vi "Main Editor UI.vi"() -> ()   [LabVIEW 2015, in "SystemLink editor node.lvclass"]
doc: "This is the main view for configuration the behavior of a module in the DCAF standard editor."
uses:
  SystemLink editor node.lvclass
  <vilib>/NI/Configuration Framework/Node/NodeRef.ctl
  <vilib>/NI/Configuration Framework/Node/NISE_CEF_Node.lvclass
  <vilib>/NI/AMC/Message Queue.ctl
  <vilib>/NI/AMC/Message.ctl
  <vilib>/NI/Tools/Keyed Array/KeyedArray.ctl
  <vilib>/NI/Configuration Framework/Node/UserEventRef.ctl
  <vilib>/NI/Configuration Framework/Controls/EventCluster.ctl
  <vilib>/NI/DCAF UI Toolkit/Controls/Configure.ctl
  <vilib>/NI/DCAF UI Toolkit/Controls/Add.ctl
  <vilib>/NI/DCAF UI Toolkit/Controls/Remove.ctl
  <vilib>/NI/Configuration Framework/Node/StopEvent.ctl
  <vilib>/NI/Configuration Framework/Node/RefreshUIEvent.ctl
  <vilib>/NI/Configuration Framework/Node/CacheState.ctl
  <vilib>/NI/Configuration Framework/Node/NodeChangeEvent.ctl
  module/configuration/Permissions Enum.ctl
  <vilib>/NI/DCAF/Tag Editor Core/Table API/Available Tag Menu/channel action event.ctl
  <vilib>/NI/DCAF/Tag Editor Core/Table API/Available Tag Menu/dialog output action.ctl
  <vilib>/NI/Tag Bus Module Framework/channel/TBM channel.lvclass
  <vilib>/NI/Tag Bus/tag/tag descriptor.lvclass
  <vilib>/NI/DCAF/Tag Editor Core/Table API/Table Manager/Call Back Ref Type Def.ctl
  <vilib>/NI/DCAF/Tag Editor Core/Configuration Editor/Classes/Engine Parent/Engine Parent Editor Node.lvclass
  <vilib>/NI/DCAF/Tag Editor Core/Configuration Editor/Classes/Module editor node/module editor node.lvclass
  <vilib>/NI/DCAF UI Toolkit/Controls/Import.ctl
  <vilib>/NI/DCAF UI Toolkit/Controls/Export.ctl
  module/configuration/Data Tag Type.ctl
  <vilib>/NI/DCAF/Tag Editor Core/Table API/Table Manager/references.ctl
  module/configuration/SystemLink configuration.lvclass
  module/configuration/SystemLink configuration.lvclass/SystemLink configuration.ctl
  <vilib>/Utility/miscctls.llb/LVPositionTypeDef.ctl
  module/configuration/Read Connection Configuration.vi
  module/configuration/Read Prepend Minion ID.vi
  <vilib>/NI/Configuration Framework/serializable configuration/NISE_CEF_serializable configuration.lvclass
  <vilib>/NI/DCAF/Tag Editor Core/Table API/Listbox/Multi Column Listbox.lvclass
  <vilib>/NI/Configuration Framework/NISE_CEF_TreeControl.lvlib
  <vilib>/NI/Tools/Keyed Array/Tools_KeyedArray.lvlib
  <vilib>/NI/AMC/AMC.lvlib
  <vilib>/NI/DCAF/Tag Editor Core/Table API/Table Manager.lvlib
  <vilib>/NI/DCAF/Tag Editor Core/Table API/Table Manager/Table Manager.lvclass
  <vilib>/NI/DCAF UI Toolkit/Controls/DCAF UI Elements.lvlib
panel:
  in  "Data Type":T1
  in  "user event out":refnum<user-event>
  in  "Permissions":T2
  in  "node change":T3
  in  "cache state":T4
  in  "refresh UI":T5
  in  "stop event":T6
  in  "Tab Control":T7(tab)
  in  "PrependMinionID":bool=TRUE caption="Prepend Tags With Minion ID?"
  in  "Remove Button":T8
  in  "Add Button":T9
  in  "Table":i32(listbox)
  in  "settings":T10
  in  "Configuration":T11={"Configuration ID"="", "HTTP"={"Verify Server?"=TRUE, "Server URL"="", "CA Certificate File"="", "User Info"={"Username"="", "Password"=""}, "API Key"=""}}
  in  "Connection Type":T12(ring)
  in  "Export":T13
  in  "Import":T14
  in  "user event":T15
  in  "main queue":T16
  in  "node ref":T17
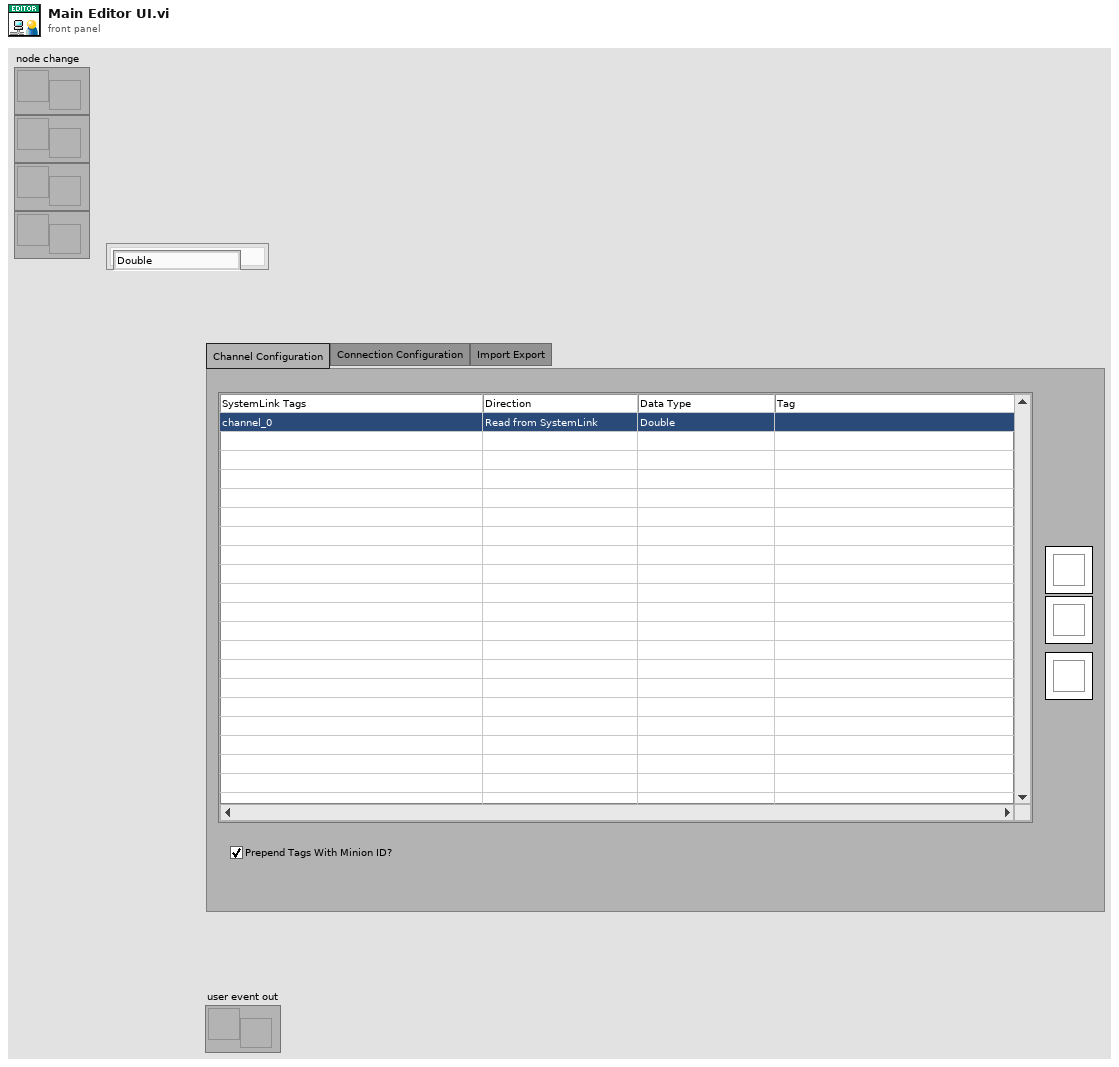
[diagram p1: front panel]
types:
  T1 = typedef "SystemLink configuration.lvclass/Data Tag Type.ctl" = enum16{"Double", "Single", "I32", "I16", "I8", "U64", "U32", "U16", "U8", "Boolean", "String", "Timestamp"}
  T2 = typedef "SystemLink configuration.lvclass/Permissions Enum.ctl" = enum16{"Read from SystemLink", "Write to SystemLink"}
  T3 = typedef "NISE_CEF_Node.lvclass/NodeChangeEvent.ctl" = refnum<user-event>
  T4 = typedef "NISE_CEF_Node.lvclass/CacheState.ctl" = refnum<user-event>
  T5 = typedef "NISE_CEF_Node.lvclass/RefreshUIEvent.ctl" = refnum<user-event>
  T6 = typedef "NISE_CEF_Node.lvclass/StopEvent.ctl" = refnum<user-event>
  T7 = enum32{"Channel Configuration", "Connection Configuration", "Import Export"}
  T8 = typedef "DCAF UI Elements.lvlib/Remove.ctl" = bool
  T9 = typedef "DCAF UI Elements.lvlib/Add.ctl" = bool
  T10 = typedef "DCAF UI Elements.lvlib/Configure.ctl" = bool
  T11 = cluster{"Configuration ID":string, "HTTP":cluster{"Verify Server?":bool, "Server URL":string, "CA Certificate File":string, "User Info":cluster{"Username":string, "Password":string}, "API Key":string}}
  T12 = enum16{"AMQP", "HTTP", "API Key (SystemLink Cloud)"}
  T13 = typedef "DCAF UI Elements.lvlib/Export.ctl" = bool
  T14 = typedef "DCAF UI Elements.lvlib/Import.ctl" = bool
  T15 = typedef "NISE_CEF_Node.lvclass/UserEventRef.ctl" = refnum<user-event>
  T16 = typedef "AMC.lvlib/Message Queue.ctl" = refnum<queue>
  T17 = typedef "NISE_CEF_Node.lvclass/NodeRef.ctl" = refnum<data-value>
  T18 = typedef "Table Manager.lvlib/Table Manager.lvclass/references.ctl" = cluster{"stop event":T6, "refresh UI":T5, "cache state":T4, "node change":T3, "user event out":refnum<user-event>, "main queue":T16, "user event":T15}
  T19 = typedef "LVPositionTypeDef.ctl" = cluster{"Left":i32, "Top":i32}
  T20 = typedef "Table Manager.lvlib/Table Manager.lvclass/object ref.ctl" = cluster{"engine":refnum<data-value>, "Node Ref":refnum<data-value>}
  T21 = typedef "Table Manager.lvlib/Column.lvclass/Column Descriptor.ctl" = cluster{"name":string, "caption":string, "Column Type":T22, "Params":string, "AutoSizeMode":i32, "FillWeight":sgl, "MinWidth":u32, "tooltip":string, "Enum Reference":refnum<vi>, "Channel suffix":string, "Read Only":bool, "Call Back VI":T23, "DT Dependency":i32, "name dependency":i32, "data type":T24, "Custom Column":refnum<class "Column.lvclass">}
  T22 = typedef "Table Manager.lvlib/Column.lvclass/Column Type.ctl" = enum16{"String", "Mapping", "Enum", "Custom"}
  T23 = typedef "Table Manager.lvlib/Table Manager.lvclass/Call Back Ref Type Def.ctl" = refnum<vi>
  T24 = typedef "tag bus.lvlib/tag descriptor.lvclass/Data Type.ctl" = enum16{"Double", "Single", "I64", "I32", "I16", "I8", "U64", "U32", "U16", "U8", "Boolean", "String", "Array of Double", "Array of Single", "Array of I64", "Array of I32", "Array of I16", "Array of I8", "Array of U64", "Array of U32", "Array of U16", "Array of U8", "Array of Boolean", "Array of String"}
  T25 = typedef "SystemLink configuration.lvclass/Connection Configuration.ctl" = cluster{"Connection Type":T26, "AMQP":cluster{"Configuration ID":string}, "HTTP":cluster{"Verify Server?":bool, "Server URL":string, "CA Certificate File":string, "User Info":cluster{"Username":string, "Password":string}, "API Key":string}}
  T26 = typedef "SystemLink configuration.lvclass/Connection Type.ctl" = enum16{"AMQP", "HTTP", "API Key (SystemLink Cloud)"}
  T27 = cluster{"Verify Server?":bool, "Server URL":string, "CA Certificate File":string, "User Info":cluster{"Username":string, "Password":string}, "API Key":string}
  T28 = typedef "Table Manager.lvlib/Table Manager.lvclass/Table Events.ctl" = cluster{"Menu Selection":refnum<user-event>}
  T29 = enum8{"Enabled", "Disabled", "Disabled and Grayed Out"}
  T30 = cluster{"AMQP Specific":refnum<vi>, "HTTP Generic":refnum<vi>, "HTTP Specific":refnum<vi>, "API Key Specific":refnum<vi>}
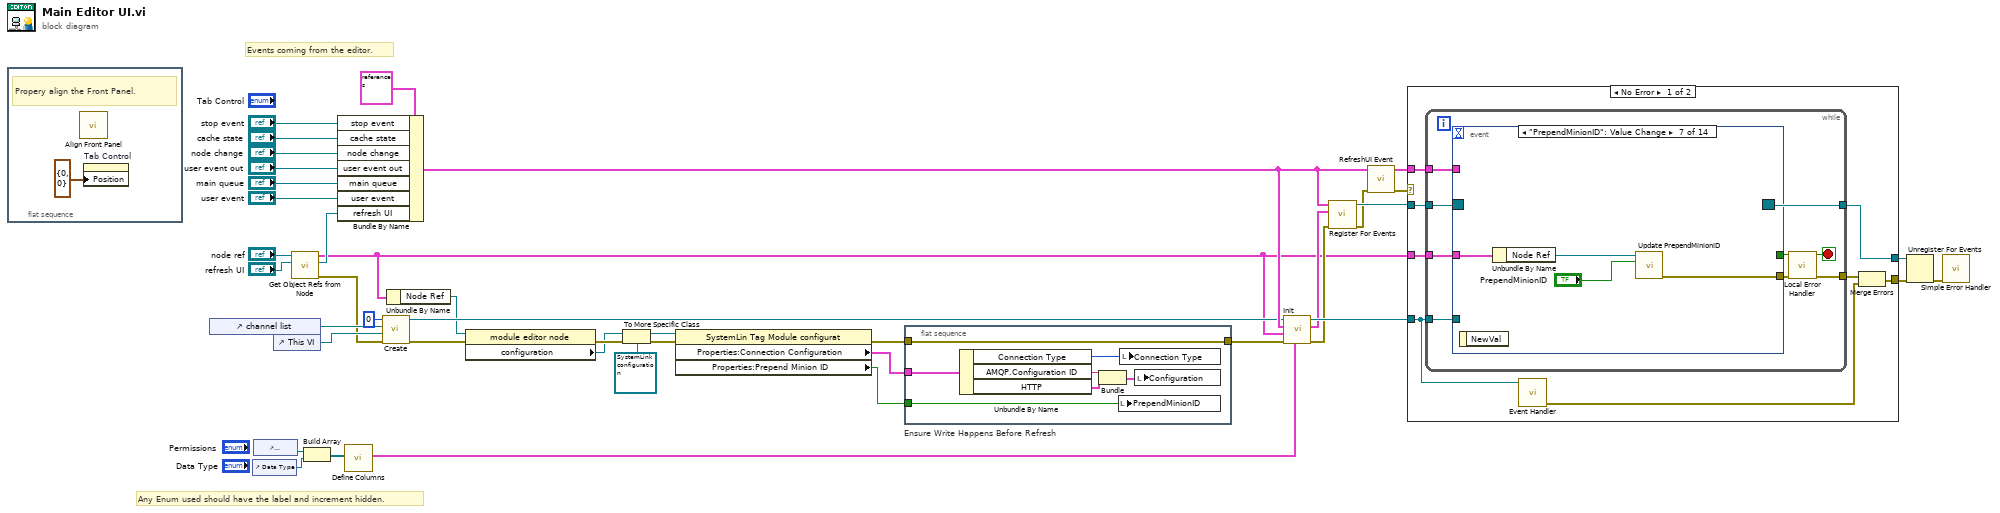
[diagram p0: block diagram]
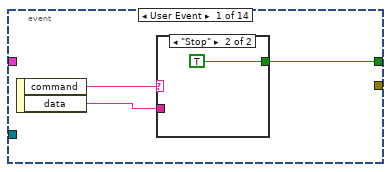
[diagram p2: hidden frame]
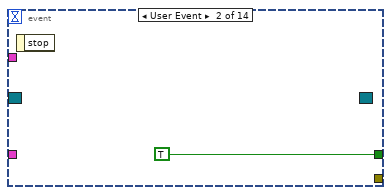
[diagram p4: hidden frame]
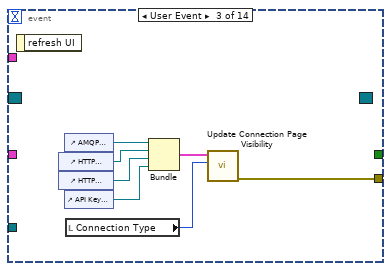
[diagram p5: hidden frame]
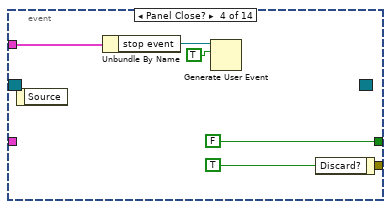
[diagram p6: hidden frame]
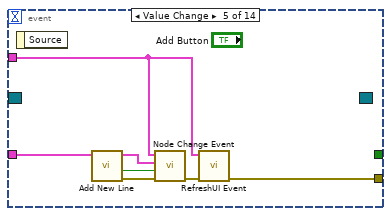
[diagram p7: hidden frame]
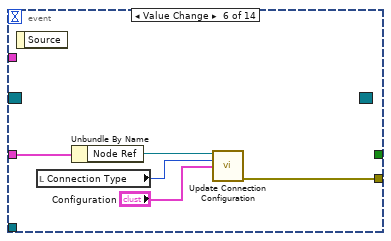
[diagram p8: hidden frame]
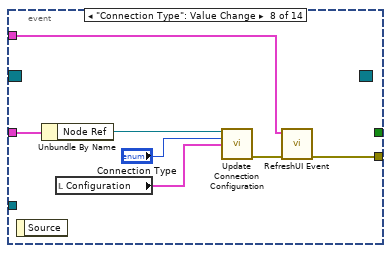
[diagram p9: hidden frame]
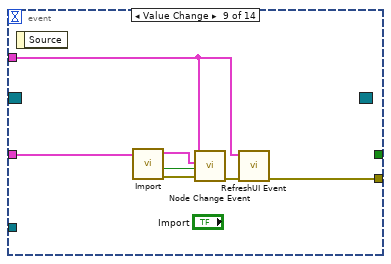
[diagram p10: hidden frame]
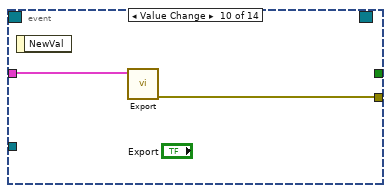
[diagram p11: hidden frame]
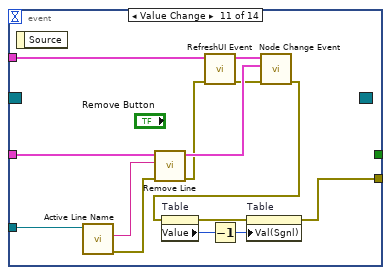
[diagram p12: hidden frame]
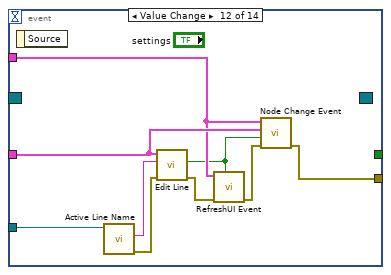
[diagram p13: hidden frame]
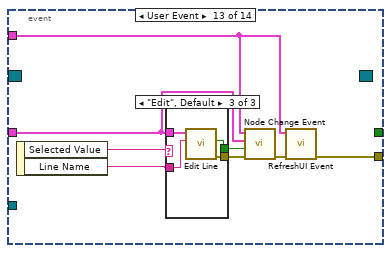
[diagram p14: hidden frame]
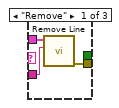
[diagram p15: hidden frame]
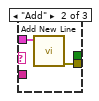
[diagram p16: hidden frame]
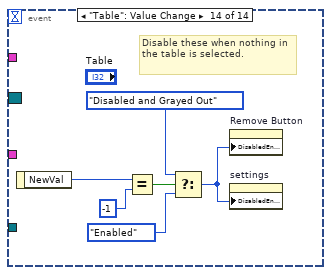
[diagram p17: hidden frame]
diagram:
  # "Any Enum used should have the label and increment hidden."
  # "Events coming from the editor."
  n1 = flat-sequence {
    frame #0 {
      # "Propery align the Front Panel."
      n2 = call <vilib>:"Align Front Panel.vi"() -> ()  [unwired: 10 in, 2 out]
      n3 = property on="Tab Control" class="TabCtl (strict)"("Position"=T19 {"Left"=0, "Top"=0}) -> ()  [unwired: 2 in, 2 out]
    }
  }
  n4 = control-ref of="channel list"() -> (w20:refnum<vi>)
  n5 = control-ref of="Data Type"() -> (w12:refnum<vi>)
  n6 = control-ref of="Permissions"() -> (w28:refnum<vi>)
  n7 = control-ref of="This VI"() -> (w18:refnum<vi>)
  n8 = call "Get Object Refs from Node.vi"("Refresh UI"="refresh UI", "Data Value Reference in"="node ref") -> ("error out"=w15:errorcluster, "Refresh UI out"=w13:T5, "References"=w10:T20)  [unwired: 7 in]
  n9 = Build Array(w28, w12) -> (w27:refnum<vi>[])
  n10 = Bundle By Name(cluster=T18 {"stop event"=refnum, "refresh UI"=refnum, "cache state"=refnum, "node change"=refnum, "user event out"=refnum, "main queue"=refnum, "user event"=refnum} ("References"), "stop event"="stop event", "cache state"="cache state", "node change"="node change", "user event out"="user event out", "main queue"="main queue", "user event"="user event", "refresh UI"=w13) -> (w29:T18)
  n11 = call "Define Columns.vi"("Enum Array"=w27) -> ("Column Definition"=w31:T21[])  [unwired: 10 in]
  n12 = call <vilib>:"Create.vi"("error in (no error)"=w15, "Top VI"=w18, "Listbox"=w20, "Index"=0) -> ("error out"=w16:errorcluster, "reference out"=w17:refnum<class "Multi Column Listbox.lvclass">)  [unwired: 6 in]
  n13 = Unbundle By Name(w10) -> ("Node Ref"=w9:refnum<data-value>)
  n14 = property class="module editor node"(reference=w9, error in=w16) -> (error out=w11:errorcluster, "configuration"=w7:refnum<class "NISE_CEF_serializable configuration.lvclass">)  [unwired: 1 out]
  n15 = To More Specific Class(target class=refnum<class "SystemLink configuration.lvclass"> refnum ("SystemLin Tag Module configuration"), reference=w7, error in=w11) -> (specific class reference=w5:refnum<class "SystemLink configuration.lvclass">, error out=w8:errorcluster)
  n16 = property class="SystemLin Tag Module configurat"(reference=w5, error in=w8) -> (error out=w3:errorcluster, "Properties:Connection Configuration"=w4:T25, "Properties:Prepend Minion ID"=w1:bool)  [unwired: 1 out]
  n17 = flat-sequence "Ensure Write Happens Before Refresh" {
    tunnel: w4 -> [w50]
    tunnel: w3 -> [w48]
    tunnel: [w48] -> w2
    tunnel: w1 -> [w44]
    frame #0 {
      n18 = Unbundle By Name(w50) -> ("Connection Type"=w49:T26, "AMQP.Configuration ID"=w46:string, "HTTP"=w45:T27)
      n19 = Bundle("Configuration ID"=w46, "HTTP"=w45) -> (w47:T11)  [unwired: 1 in]
      n20 = local write "PrependMinionID"(w44) -> ()
      n21 = local write "Connection Type"(w49) -> ()
      n22 = local write "Configuration"(w47) -> ()
    }
  }
  n23 = call-dynamic "Init.vi"("Column Descriptors"=w31, "error in (no error)"=w2, "Node object refs"=w10, "Event References"=w29, "Multi Column Listbox in"=w17) -> ("error out"=w22:errorcluster, "Table Events"=w21:T28, "Multi Column Listbox out"=w26:refnum<class "Multi Column Listbox.lvclass">)  [unwired: 4 in]
  n24 = call "Register For Events.vi"("error in"=w22, "Table Events"=w21, "References"=w29) -> ("error out"=w24:errorcluster, "Event Registration Refnum"=w32:refnum<event-registration>)  [unwired: 7 in]
  n25 = call "RefreshUI Event.vi"("error in (no error)"=w24, "References in"=w29) -> ("error out"=w23:errorcluster, "References out"=w30:T18)  [unwired: 8 in]
  n26 = case shown="No Error" w23 {
    selector: w23 -> [_ w162]
    tunnel: w32 -> [w58 w161]
    tunnel: [w57 w161] -> w42
    tunnel: [w51 w162] -> w41
    tunnel: w30 -> [w56 _]
    tunnel: w10 -> [w55 _]
    tunnel: w26 -> [w54 _]
    frame No Error {
      n27 = while {
        tunnel: w58 -> [w67]
        tunnel: [w66] -> w57
        tunnel: [w63] -> w52
        tunnel: w56 -> [w61]
        tunnel: w55 -> [w60]
        tunnel: w54 -> [w59]
        stop <- w65 stop-if-true
        n28 = event shown="[6] \"PrependMinionID\": Value Change" {
          selector: w67 -> [_ _ _ _ _ _ _ _ _ _ _ _ _ _]
          dyn-events: [_ _ _ _ _ _ _ _ _ _ _ _ _ _] -> w66
          timeout: _ -> [_ _ _ _ _ _ _ _ _ _ _ _ _ _]
          tunnel: [w70 TRUE _ FALSE _ _ _ _ _ _ _ _ _ _] -> w64
          tunnel: [_ _ w73 _ w85 w93 w98 w102 w112 w115 w117 w137 w143 _] -> w62
          tunnel: w61 -> [_ _ _ w81 w89 _ _ w101 w109 _ w128 w132 w139 _]
          tunnel: w60 -> [_ _ _ _ w90 w95 w97 w105 w111 w114 w127 w135 w140 _]
          tunnel: w59 -> [_ _ _ _ _ _ _ _ _ _ w123 w136 _ _]
          event User Event {
            n29 = event-data() -> ("command"=w69:string, "data"=w68:string)  [unwired: 1 in]
            n30 = case shown="\"Stop\"" w69 {
              tunnel: [_ TRUE] -> w70
              tunnel: w68 -> [_ _]
              frame Default {
              }
              frame "Stop" {
              }
            }
          }
          event User Event {
            n31 = event-data() -> ()  [unwired: 1 in, 1 out]
          }
          event User Event {
            n32 = event-data() -> ()  [unwired: 1 in, 1 out]
            n33 = control-ref of="HTTP Generic"() -> (w78:refnum<vi>)
            n34 = control-ref of="HTTP Specific"() -> (w77:refnum<vi>)
            n35 = control-ref of="AMQP Specific"() -> (w79:refnum<vi>)
            n36 = control-ref of="API Key Specific"() -> (w76:refnum<vi>)
            n37 = local read "Connection Type"() -> (w74:T12)
            n38 = Bundle("AMQP Specific"=w79, "HTTP Generic"=w78, "HTTP Specific"=w77, "API Key Specific"=w76) -> (w75:T30)  [unwired: 1 in]
            n39 = call "Update Connection Page Visibility.vi"("Connection Type"=w74, "Config References"=w75) -> ("error out"=w73:errorcluster)  [unwired: 9 in]
          }
          event Panel Close? {
            n40 = event-data() -> ()  [unwired: 1 in, 1 out]
            n41 = Unbundle By Name(w81) -> ("stop event"=w80:T6)
            n42 = Generate User Event(user event=w80, event data cluster=TRUE ("event data")) -> ()  [unwired: 2 in, 2 out]
            n43 = event-data("Discard?"=TRUE) -> ()  [unwired: 1 in, 1 out]
          }
          event Value Change {
            n44 = event-data() -> ()  [unwired: 1 in, 1 out]
            n45 = call "Add New Line.vi"("objects"=w90) -> ("error out"=w88:errorcluster, "success"=w86:bool)  [unwired: 8 in, 1 out]
            n46 = call "Node Change Event.vi"("error in (no error)"=w88, "Send (T)"=w86, "objects"=w90, "References in"=w89) -> ("error out"=w87:errorcluster)  [unwired: 7 in]
            n47 = call "RefreshUI Event.vi"("error in (no error)"=w87, "References in"=w89) -> ("error out"=w85:errorcluster)  [unwired: 8 in, 1 out]
          }
          event "Configuration.HTTP", "Configuration.Configuration ID": Value Change {
            n48 = event-data() -> ()  [unwired: 1 in, 1 out]
            n49 = local read "Connection Type"() -> (w92:T12)
            n50 = Unbundle By Name(w95) -> ("Node Ref"=w94:refnum<data-value>)
            n51 = call "Update Connection Configuration.vi"("Data Value Reference in"=w94, "Connection Type"=w92, "Configuration"="Configuration") -> ("error out"=w93:errorcluster)  [unwired: 12 in]
          }
          event "PrependMinionID": Value Change {
            n52 = event-data() -> ()  [unwired: 1 in, 1 out]
            n53 = Unbundle By Name(w97) -> ("Node Ref"=w96:refnum<data-value>)
            n54 = call "Update PrependMinionID.vi"("PrependMinionID"="PrependMinionID", "Data Value Reference in"=w96) -> ("error out"=w98:errorcluster)  [unwired: 9 in]
          }
          event "Connection Type": Value Change {
            n55 = event-data() -> ()  [unwired: 1 in, 1 out]
            n56 = Unbundle By Name(w105) -> ("Node Ref"=w106:refnum<data-value>)
            n57 = local read "Configuration"() -> (w100:T11)
            n58 = call "Update Connection Configuration.vi"("Data Value Reference in"=w106, "Connection Type"="Connection Type", "Configuration"=w100) -> ("error out"=w103:errorcluster)  [unwired: 12 in]
            n59 = call "RefreshUI Event.vi"("error in (no error)"=w103, "References in"=w101) -> ("error out"=w102:errorcluster)  [unwired: 8 in, 1 out]
          }
          event Value Change {
            n60 = event-data() -> ()  [unwired: 1 in, 1 out]
            n61 = call "Import.vi"("Objects in"=w111) -> ("error out"=w108:errorcluster, "Update"=w107:bool, "Objects out"=w110:T20)  [unwired: 8 in]
            n62 = call "Node Change Event.vi"("error in (no error)"=w108, "Send (T)"=w107, "objects"=w110, "References in"=w109) -> ("error out"=w113:errorcluster)  [unwired: 7 in]
            n63 = call "RefreshUI Event.vi"("error in (no error)"=w113, "References in"=w109) -> ("error out"=w112:errorcluster)  [unwired: 8 in, 1 out]
          }
          event Value Change {
            n64 = event-data() -> ()  [unwired: 1 in, 1 out]
            n65 = call "Export.vi"("Objects"=w114) -> ("error out"=w115:errorcluster)  [unwired: 10 in]
          }
          event Value Change {
            n66 = event-data() -> ()  [unwired: 1 in, 1 out]
            n67 = call-dynamic "Active Line Name.vi"("Multi Column Listbox in"=w123) -> ("error out"=w121:errorcluster, "Active Line Name"=w122:string)  [unwired: 8 in, 1 out]
            n68 = call "Remove Line.vi"("error in"=w121, "Active Line Name"=w122, "Objects"=w127) -> ("error out"=w124:errorcluster)  [unwired: 8 in]
            n69 = call "RefreshUI Event.vi"("error in (no error)"=w124, "References in"=w128) -> ("error out"=w126:errorcluster, "References out"=w125:T18)  [unwired: 8 in]
            n70 = call "Node Change Event.vi"("error in (no error)"=w126, "objects"=w127, "References in"=w125) -> ("error out"=w118:errorcluster)  [unwired: 8 in]
            n71 = property on="Table" class="MCListbox (strict)"(error in=w118) -> (error out=w116:errorcluster, "Value"=w119:i32)  [unwired: 1 in, 1 out]
            n72 = Decrement(x=w119) -> (x-1=w120:i32)
            n73 = property on="Table" class="MCListbox (strict)"(error in=w116, "Val(Sgnl)"=w120) -> (error out=w117:errorcluster)  [unwired: 1 in, 1 out]
          }
          event Value Change {
            n74 = event-data() -> ()  [unwired: 1 in, 1 out]
            n75 = call-dynamic "Active Line Name.vi"("Multi Column Listbox in"=w136) -> ("error out"=w133:errorcluster, "Active Line Name"=w134:string)  [unwired: 8 in, 1 out]
            n76 = call "Edit Line.vi"("error in"=w133, "Line Name"=w134, "References"=w135) -> ("error out"=w130:errorcluster, "change?"=w131:bool)  [unwired: 7 in]
            n77 = call "RefreshUI Event.vi"("Refresh (T)"=w131, "error in (no error)"=w130, "References in"=w132) -> ("error out"=w129:errorcluster)  [unwired: 7 in, 1 out]
            n78 = call "Node Change Event.vi"("error in (no error)"=w129, "Send (T)"=w131, "objects"=w135, "References in"=w132) -> ("error out"=w137:errorcluster)  [unwired: 7 in]
          }
          event User Event {
            n79 = event-data() -> ("Selected Value"=w145:string, "Line Name"=w142:string)  [unwired: 1 in]
            n80 = case shown="\"Edit\", Default" w145 {
              tunnel: w142 -> [w148 _ w154]
              tunnel: w140 -> [w147 w150 w153]
              tunnel: [w146 w149 w152] -> w141
              tunnel: [_ _ w151] -> w138
              frame "Remove" {
                n81 = call "Remove Line.vi"("Active Line Name"=w148, "Objects"=w147) -> ("error out"=w146:errorcluster)  [unwired: 9 in]
              }
              frame "Add" {
                n82 = call "Add New Line.vi"("objects"=w150) -> ("error out"=w149:errorcluster)  [unwired: 8 in, 2 out]
              }
              frame "Edit", Default {
                n83 = call "Edit Line.vi"("Line Name"=w154, "References"=w153) -> ("error out"=w152:errorcluster, "change?"=w151:bool)  [unwired: 8 in]
              }
            }
            n84 = call "Node Change Event.vi"("error in (no error)"=w141, "Send (T)"=w138, "objects"=w140, "References in"=w139) -> ("error out"=w144:errorcluster)  [unwired: 7 in]
            n85 = call "RefreshUI Event.vi"("error in (no error)"=w144, "References in"=w139) -> ("error out"=w143:errorcluster)  [unwired: 8 in, 1 out]
          }
          event "Table": Value Change {
            # "Disable these when nothing in the table is selected."
            n86 = event-data() -> ("NewVal"=w160:i32)  [unwired: 1 in]
            n87 = Equal?(x=w160, y=-1) -> (x = y?=w158:bool)
            n88 = Select(t=T29."Disabled and Grayed Out" ("Disabled"), s=w158, f=T29."Enabled") -> (s? t:f=w156:T29)
            n89 = property on="Remove Button" class="Bool"("DisabledEnum"=w156) -> ()  [unwired: 2 in, 2 out]
            n90 = property on="settings" class="Bool"("DisabledEnum"=w156) -> ()  [unwired: 2 in, 2 out]
          }
        }
        n91 = call "Local Error Handler.vi"("error in"=w62, "Stop in"=w64) -> ("error out"=w63:errorcluster, "Stop out"=w65:bool)  [unwired: 8 in]
      }
      n92 = call-dynamic "Event Handler.vi"("Listbox in"=w54) -> ("error out"=w53:errorcluster)  [unwired: 9 in, 1 out]
      n93 = Merge Errors(w52, w53) -> (w51:errorcluster)
    }
    frame Error {
    }
  }
  n94 = Unregister For Events(event registration refnum=w42, error in=w41) -> (error out=w40:errorcluster)
  n95 = call <vilib>:"Simple Error Handler.vi"("error in (no error)"=w40) -> ()  [unwired: 4 in, 5 out]
